vi "Rename State.vi"(5 "Category":string, 7 "State":string, 8 "error in (no error)":errorcluster, 9 "New State":string, 10 "New Category (\"\": Use Existing)":string, 11 "JKI SM in":refnum<class "JKI SM.lvclass">) -> (0 "error out":errorcluster, 1 "New Frame Names":string[](array[string]), 2 "Old Frame Names":string[](array[string]), 3 "JKI SM out":refnum<class "JKI SM.lvclass">)   [LabVIEW 2020, in "JKI State Machine API.lvlib" / "JKI SM.lvclass"]
uses:
  JKI SM.lvclass
  JKI SM.lvclass/JKI SM.ctl
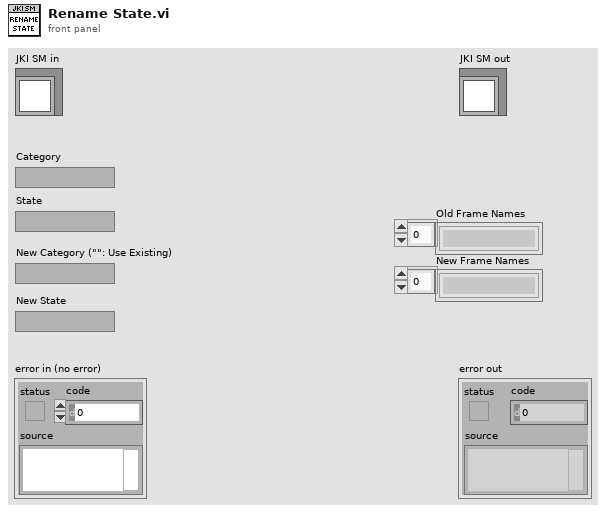
[diagram p1: front panel]
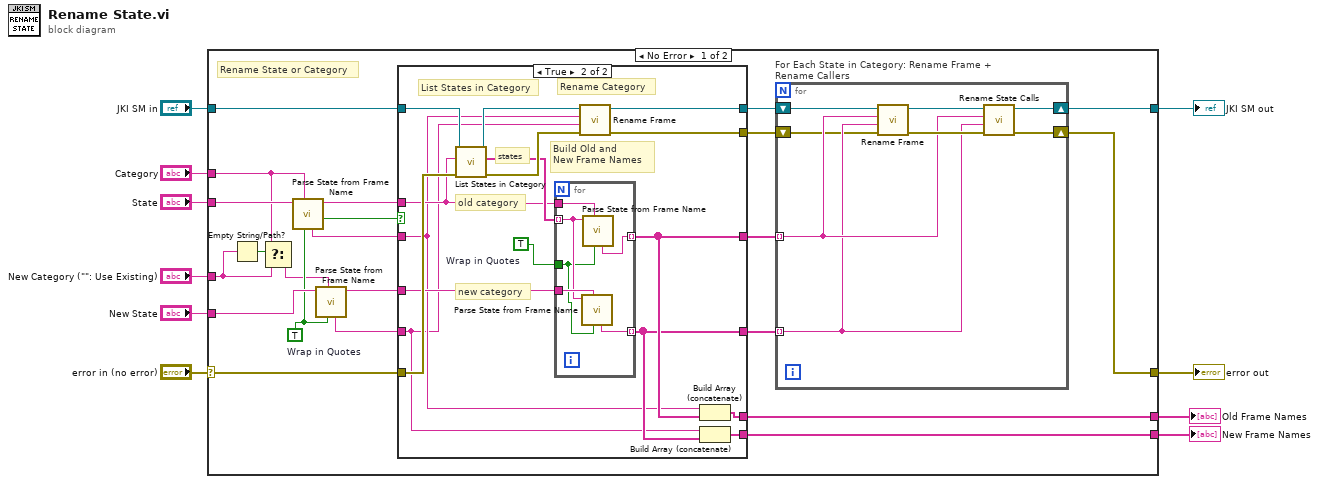
[diagram p0: block diagram]
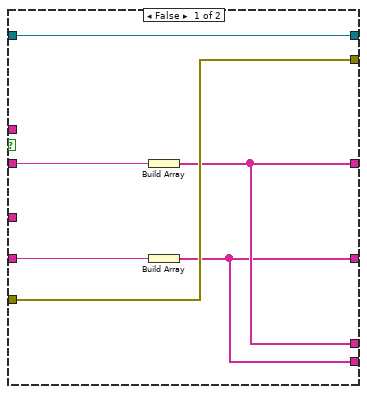
[diagram p2: hidden frame]
diagram:
  n1 = case shown="No Error" "error in (no error)" {
    selector: "error in (no error)" -> [w19 w70]
    tunnel: [w32 w70] -> w9
    tunnel: [w24 w69] -> w7
    tunnel: "JKI SM in" -> [w22 w69]
    tunnel: "Category" -> [w27 _]
    tunnel: "State" -> [w31 _]
    tunnel: "New Category (\"\": Use Existing)" -> [w26 _]
    tunnel: "New State" -> [w30 _]
    tunnel: [w12 _] -> w2
    tunnel: [w11 _] -> w1
    frame No Error {
      w29 = TRUE  # Wrap in Quotes
      # "Rename State or Category"
      n2 = Empty String/Path?(string/path=w26) -> (empty?=w28:bool)
      n3 = Select(t=w27, s=w28, f=w26) -> (s? t:f=w25:string)
      n4 = call "Parse State from Frame Name.vi"("Wrap in Quotes? (FALSE)"=w29, "Category (Optional)"=w27, "Frame or State Name"=w31) -> ("is a Category Frame?"=w23:bool, "Category Name"=w17:string, "\"Category: State\" String"=w20:string)  [unwired: 3 in, 3 out]
      n5 = call "Parse State from Frame Name.vi"("Wrap in Quotes? (FALSE)"=w29, "Category (Optional)"=w25, "Frame or State Name"=w30) -> ("Category Name"=w16:string, "\"Category: State\" String"=w15:string)  [unwired: 3 in, 4 out]
      n6 = case shown="True" w23 {
        tunnel: w22 -> [w46 w61]
        tunnel: [w46 w62] -> w21
        tunnel: w20 -> [w44 w48]
        tunnel: w15 -> [w43 w47]
        tunnel: w19 -> [w45 w58]
        tunnel: [w45 w57] -> w18
        tunnel: w17 -> [_ w54]
        tunnel: w16 -> [_ w55]
        tunnel: [w42 w52] -> w14
        tunnel: [w41 w51] -> w13
        tunnel: [w42 w50] -> w12
        tunnel: [w41 w49] -> w11
        frame False {
          n7 = Build Array(w44) -> (w42:string[])
          n8 = Build Array(w43) -> (w41:string[])
        }
        frame True {
          w53 = TRUE  # Wrap in Quotes
          # "states"
          # "new category"
          # "old category"
          # "Build Old and\nNew Frame Names"
          # "Rename Category"
          # "List States in Category"
          n9 = call "List States in Category.vi"("error in (no error)"=w58, "Category"=w54, "JKI SM in"=w61) -> ("error out"=w59:errorcluster, "States"=w56:string[], "JKI SM out"=w60:refnum<class "JKI SM.lvclass">)  [unwired: 4 in, 2 out]
          n10 = for {
            tunnel: w56 -> [w66] mode=indexing
            tunnel: w54 -> [w68]
            tunnel: w55 -> [w67]
            tunnel: [w65] -> w51 mode=indexing
            tunnel: [w64] -> w52 mode=indexing
            tunnel: w53 -> [w63]
            n11 = call "Parse State from Frame Name.vi"("Wrap in Quotes? (FALSE)"=w63, "Category (Optional)"=w67, "Frame or State Name"=w66) -> ("\"Category: State\" String"=w65:string)  [unwired: 3 in, 5 out]
            n12 = call "Parse State from Frame Name.vi"("Wrap in Quotes? (FALSE)"=w63, "Category (Optional)"=w68, "Frame or State Name"=w66) -> ("\"Category: State\" String"=w64:string)  [unwired: 3 in, 5 out]
          }
          n13 = call "Rename Frame.vi"("error in (no error)"=w59, "New Frame Name (with quotes)"=w47, "Old Frame Name (with quotes)"=w48, "JKI SM in"=w60) -> ("error out"=w57:errorcluster, "JKI SM out"=w62:refnum<class "JKI SM.lvclass">)  [unwired: 6 in]
          n14 = Build Array (concatenate)(w48, w52) -> (w50:string[])
          n15 = Build Array (concatenate)(w47, w51) -> (w49:string[])
        }
      }
      n16 = for "For Each State in Category: Rename Frame + Rename Callers" {
        tunnel: w14 -> [w35] mode=indexing
        tunnel: w13 -> [w34] mode=indexing
        shift-right: [w37] -> w24
        shift-left: w21 -> [w36]
        shift-right: [w40] -> w32
        shift-left: w18 -> [w33]
        n17 = call "Rename Frame.vi"("error in (no error)"=w33, "New Frame Name (with quotes)"=w34, "Old Frame Name (with quotes)"=w35, "JKI SM in"=w36) -> ("error out"=w39:errorcluster, "JKI SM out"=w38:refnum<class "JKI SM.lvclass">)  [unwired: 6 in]
        n18 = call "Rename State Calls.vi"("error in (no error)"=w39, "New State Name"=w34, "Old State Name"=w35, "JKI SM in"=w38) -> ("error out"=w40:errorcluster, "JKI SM out"=w37:refnum<class "JKI SM.lvclass">)  [unwired: 6 in]
      }
    }
    frame Error {
    }
  }
  "error out" <- w9
  "JKI SM out" <- w7
  "Old Frame Names" <- w2
  "New Frame Names" <- w1
